vi "Load Config.vi"(6 "Constants":refnum<class "Sequence Constants.lvclass">, 8 "error in (no error)":refnum<class "MultiErrors.lvclass">, 10 "Config Element":refnum<class "Config Element.lvclass">, 11 "HighLimit Condition Config in":refnum<class "HighLimit Condition Config.lvclass">) -> (0 "error out":refnum<class "MultiErrors.lvclass">, 3 "HighLimit Condition Config out":refnum<class "HighLimit Condition Config.lvclass">)   [LabVIEW 2020, in "VolatusSeqConfig.lvlib" / "HighLimit Condition Config.lvclass"]
uses:
  HighLimit Condition Config.lvclass
  VolatusErrorUtilities/MultiErrors/MultiErrors.lvclass
  lv-cdm/CDM-Config/Config Element/Config Element.lvclass
  Sequence Constants/Sequence Constants.lvclass
  HighLimit Condition Config.lvclass/HighLimit Condition Config.ctl
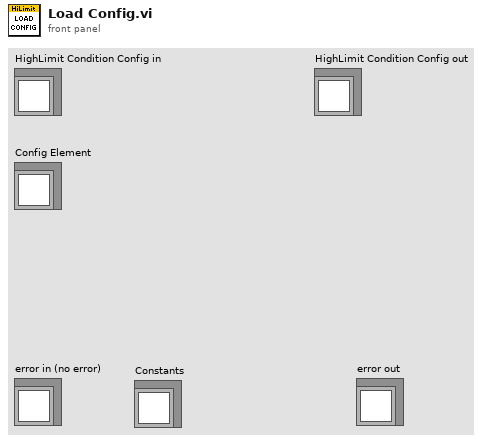
[diagram p1: front panel]
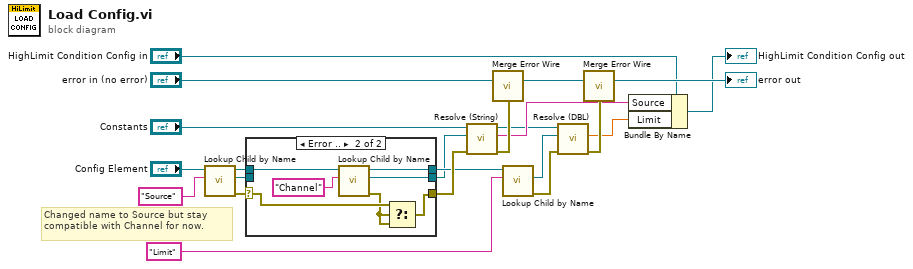
[diagram p0: block diagram]
diagram:
  # "Changed name to Source but stay compatible with Channel for now."
  n1 = call "Lookup Child by Name.vi"("Name"="Source", "Config Element in"="Config Element") -> ("error out"=w2:errorcluster, "Child"=w1:refnum<class "Config Element.lvclass">, "Config Element out"=w4:refnum<class "Config Element.lvclass">)  [unwired: 6 in, 1 out]
  n2 = case shown="Error .." w2 {
    selector: w2 -> [w23 w28]
    tunnel: [w23 w26] -> w22
    tunnel: [w25 w31] -> w16
    tunnel: [w24 w30] -> w14
    tunnel: w4 -> [w25 w29]
    tunnel: w1 -> [w24 _]
    frame No Error {
    }
    frame Error {
      n3 = call "Lookup Child by Name.vi"("Name"="Channel", "Config Element in"=w29) -> ("error out"=w27:errorcluster, "Child"=w30:refnum<class "Config Element.lvclass">, "Config Element out"=w31:refnum<class "Config Element.lvclass">)  [unwired: 6 in, 1 out]
      n4 = Select(t=w28, s=w27, f=w27) -> (s? t:f=w26:errorcluster)
    }
  }
  n5 = call "Resolve (String).vi"("error in (no error)"=w22, "Element"=w14, "Sequence Constants in"="Constants") -> ("error out"=w19:errorcluster, "String Value"=w12:string, "Sequence Constants out"=w6:refnum<class "Sequence Constants.lvclass">)  [unwired: 6 in]
  n6 = call "Merge Error Wire.vi"("error in (no error)"=w19, "MultiErrors in"="error in (no error)") -> ("MultiErrors out"=w8:refnum<class "MultiErrors.lvclass">)  [unwired: 13 in]
  n7 = call "Lookup Child by Name.vi"("Name"="Limit", "Config Element in"=w16) -> ("error out"=w9:errorcluster, "Child"=w11:refnum<class "Config Element.lvclass">)  [unwired: 6 in, 2 out]
  n8 = call "Resolve (DBL).vi"("error in (no error)"=w9, "Element"=w11, "Sequence Constants in"=w6) -> ("error out"=w20:errorcluster, "DBL Value"=w10:dbl)  [unwired: 6 in, 1 out]
  n9 = call "Merge Error Wire.vi"("error in (no error)"=w20, "MultiErrors in"=w8) -> ("MultiErrors out"=→"error out":refnum<class "MultiErrors.lvclass">)  [unwired: 13 in]
  n10 = Bundle By Name(cluster="HighLimit Condition Config in", "Source"=w12, "Limit"=w10) -> (→"HighLimit Condition Config out":refnum<class "HighLimit Condition Config.lvclass">)
